vi "Get Property.vi"(10 "Ctl Ref":refnum<vi>, 11 "UIP In":refnum<class "UIP Interface.lvclass">) -> (0 "Error Out":errorcluster, 3 "UIP Out":refnum<class "UIP Interface.lvclass">)   [LabVIEW 2020, in "UIM.lvlib" / "UIP Interface.lvclass"]
doc: "Overwrite this abstract method to implement child behavior for getting the property from the VI Server Control and into the UIP private data."
uses:
  UIP Interface/UIP Interface.lvclass
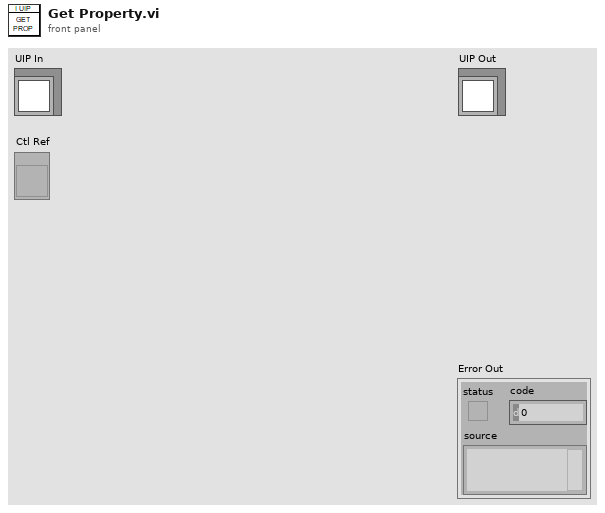
[diagram p1: front panel]
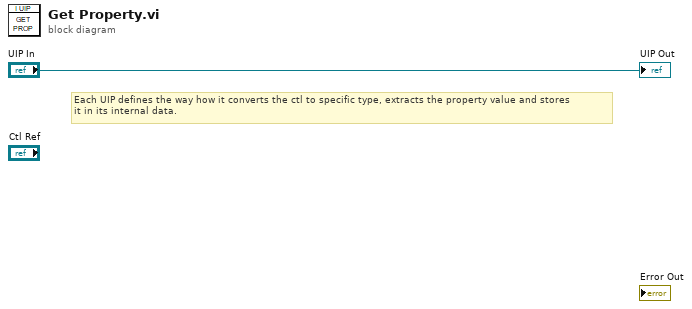
[diagram p0: block diagram]
diagram:
  # "Each UIP defines the way how it converts the ctl to specific type, extracts the property value and stores\nit in its internal data."
  "UIP Out" <- "UIP In"
